vi "Calculate Odd Parity Bit (Array).vi"(0 "Bytes":u8[](array[numeric]) format="%02x", 11 "error in (no error)":errorcluster) -> (4 "Odd Parity Bit":u8, 15 "error out":errorcluster)   [LabVIEW 2018, in "MIPI RFFE API.lvlib"]
uses:
  MIPI RFFE API.lvlib
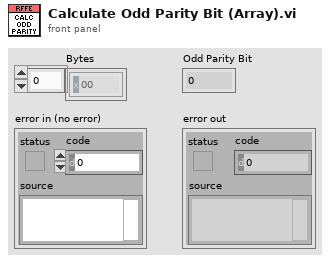
[diagram p1: front panel]
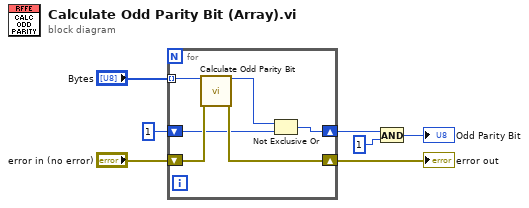
[diagram p0: block diagram]
diagram:
  n1 = for {
    shift-right: [w12] -> w6
    shift-left: "error in (no error)" -> [w13]
    tunnel: "Bytes" -> [w11] mode=indexing
    shift-right: [w8] -> w2
    shift-left: u8 1 ("y") -> [w9]
    n2 = call "Calculate Odd Parity Bit.vi"("Byte"=w11, "error in (no error)"=w13) -> ("Odd Parity Bit"=w10:u8, "error out"=w12:errorcluster)  [unwired: 12 in]
    n3 = Not Exclusive Or(1:w9, 2:w10) -> (0:w8:u8)
  }
  "error out" <- w6
  n4 = And(x=w2, y=u8 1) -> (x .and. y?=→"Odd Parity Bit":u8)
